vi "Trimming_Coil_Command.vi"() -> ()   [LabVIEW 2025]
panel:
  out "Cluster":T1
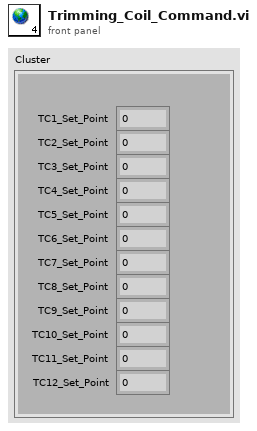
[diagram p1: front panel]
types:
  T1 = cluster{"TC1_Set_Point":dbl, "TC2_Set_Point":dbl, "TC3_Set_Point":dbl, "TC4_Set_Point":dbl, "TC5_Set_Point":dbl, "TC6_Set_Point":dbl, "TC7_Set_Point":dbl, "TC8_Set_Point":dbl, "TC9_Set_Point":dbl, "TC10_Set_Point":dbl, "TC11_Set_Point":dbl, "TC12_Set_Point":dbl}
diagram:
